vi "VIH Utility - STR - Split String to 3 Parts.vi"(9 "Position 2":i32, 10 "Position 1":i32, 11 "String":string) -> (1 "After":string, 2 "Middle":string, 3 "Before":string)   [LabVIEW 2014]
doc: "::: VI Helpeks :::\nCopyright (c) 2000-2026 Konstantin Shifershteyn. All rights reserved."
panel:
  # "VI Helpeks\nCopyright (c) 2012-2026 Konstantin Shifershteyn"
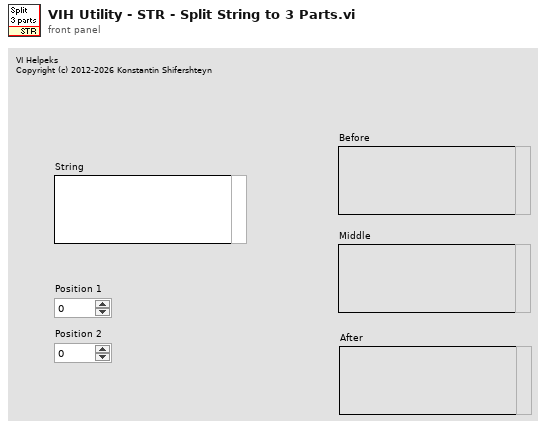
[diagram p1: front panel]
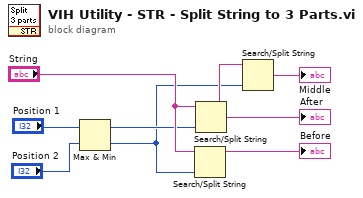
[diagram p0: block diagram]
diagram:
  n1 = Max & Min(x="Position 1", y="Position 2") -> (max(x,y)=w5:i32, min(x,y)=w1:i32)
  n2 = Search/Split String(string="String", offset (0)=w1) -> (substring before match=→"Before":string)  [unwired: 1 in, 2 out]
  n3 = Search/Split String(string="String", offset (0)=w5) -> (substring before match=w9:string, match + rest of string=→"After":string)  [unwired: 1 in, 1 out]
  n4 = Search/Split String(string=w9, offset (0)=w1) -> (match + rest of string=→"Middle":string)  [unwired: 1 in, 2 out]
